vi "OwnCompat20261012_Native_AssignConnectorTerminal.vi"() -> ()   [LabVIEW 2024]
panel:
  out "error out":errorcluster caption="错误输出"
  in  "terminal_index":u32
  in  "control_id":u32
  in  "target_path":path
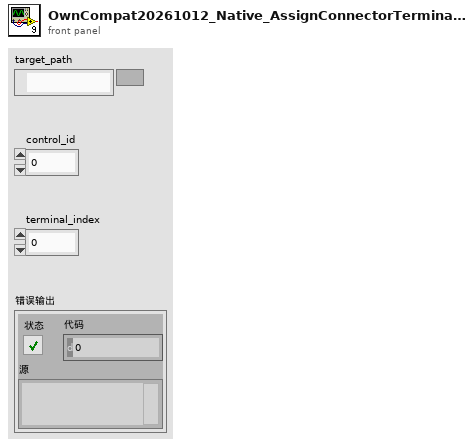
[diagram p1: front panel]
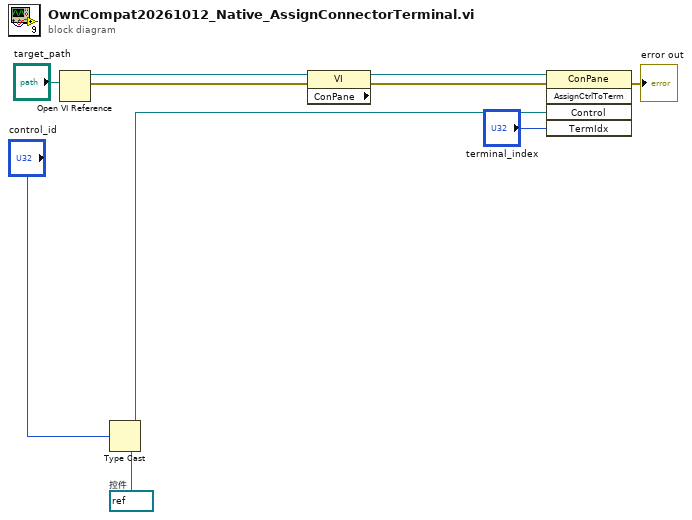
[diagram p0: block diagram]
diagram:
  w6 = refnum<vi> refnum  # 控件
  n1 = Open VI Reference ("打开VI引用")(vi path="target_path") -> (vi reference=w9:refnum<vi>, error out=w8:errorcluster)  [unwired: 5 in]
  n2 = Type Cast ("强制类型转换")(type=w6, x="control_id") -> (*(type *) &x=w3:refnum<vi>)
  n3 = property on="属性节点" class="VI"(reference=w9, error in=w8) -> (error out=w4:errorcluster, "ConPane"=w5:refnum<vi>)  [unwired: 1 out]
  n4 = invoke class="ConPane" method="AssignCtrlToTerm"(reference=w5, error in=w4, "Control"=w3, "TermIdx"="terminal_index") -> (error out=→"error out":errorcluster)  [unwired: 1 in, 4 out]
